vi "Teste_Dando_Erro.vi"() -> ()   [LabVIEW 2026]
uses:
  <vilib>/Instr/_visa.llb/VISA Configure Serial Port (Instr).vi
panel:
  out "Waveform Chart":dbl(graph)
  in  "VISA resource name":refnum<visa-resource-name>
  in  "stop":bool
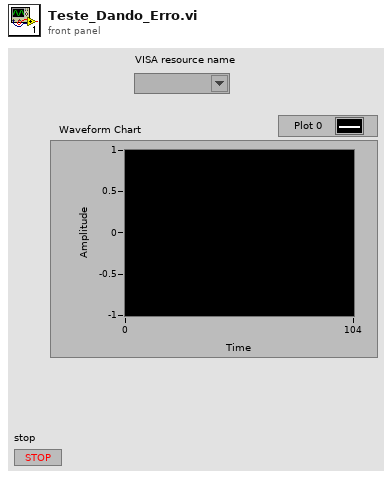
[diagram p1: front panel]
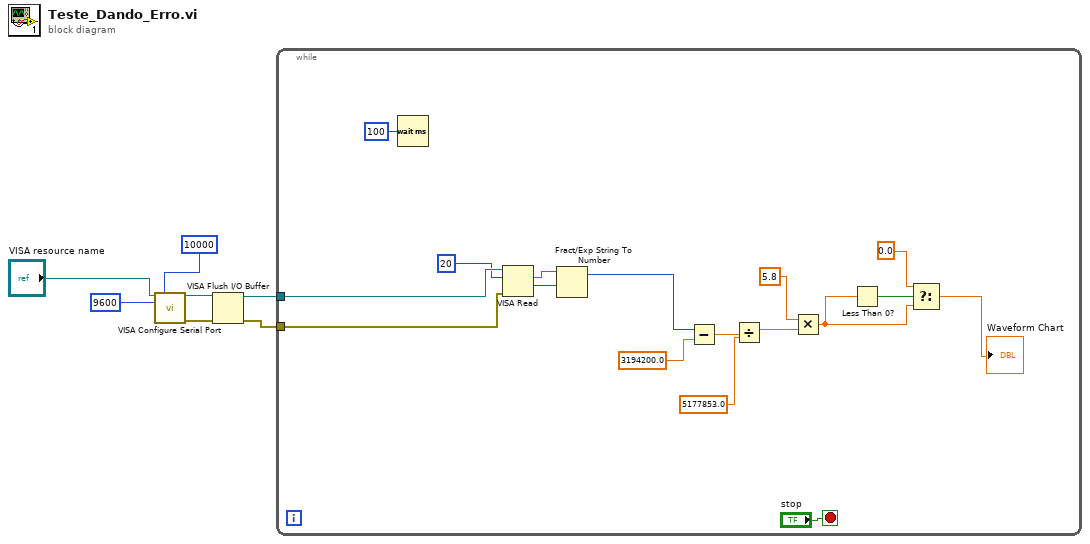
[diagram p0: block diagram]
diagram:
  n1 = call-poly "VISA Configure Serial Port"("VISA resource name"="VISA resource name", "timeout (10sec)"=u32 10000, "baud rate (9600)"=u32 9600) -> ("VISA resource name out"=w4:refnum<visa-resource-name>, "error out"=w3:errorcluster)  [unwired: 11 in]
  n2 = VISA Flush I/O Buffer(VISA resource name=w4, error in (no error)=w3) -> (VISA resource name out=w2:refnum<visa-resource-name>, error out=w1:errorcluster)  [unwired: 1 in]
  n3 = while {
    tunnel: w2 -> [w10]
    tunnel: w1 -> [w8]
    stop <- "stop" stop-if-true
    n4 = Wait (ms)(milliseconds to wait=u32 100) -> ()  [unwired: 1 out]
    n5 = VISA Read(VISA resource name=w10, byte count=u32 20, error in (no error)=w8) -> (read buffer=w12:string, return count=w13:u32)  [unwired: 2 out]
    n6 = Fract/Exp String To Number(string=w12, offset=w13) -> (offset past number=w11:i32)  [unwired: 2 in, 1 out]
    n7 = Subtract(x=w11, y=3194200.0) -> (x-y=w21:dbl)
    n8 = Divide(x=w21, y=5177853.0) -> (x/y=w19:dbl)
    n9 = Multiply(x=5.8, y=w19) -> (x*y=w15:dbl)
    n10 = Less Than 0?(x=w15) -> (x < 0?=w17:bool)
    n11 = Select(t=0.0, s=w17, f=w15) -> (s? t:f=→"Waveform Chart":dbl)
  }
